vi "Test Strict Ambiguous ISO8601 Strings.vi"(8 "error in (no error)":errorcluster) -> (0 "error out":errorcluster)   [LabVIEW 2013]
uses:
  <vilib>/Utility/file.llb/Read From Spreadsheet File (string).vi
  <vilib>/addons/_JKI Toolkits/Caraya/classes/Assert/Assert False.vi
  <vilib>/addons/_JKI Toolkits/Caraya/classes/Assert/Assert True.vi
  <vilib>/addons/_JKI Toolkits/Caraya/classes/Assert/Assert.lvclass
  <vilib>/addons/_JKI Toolkits/Caraya/classes/Test/Test.lvclass
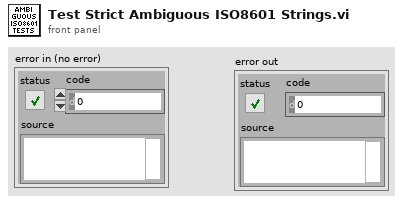
[diagram p1: front panel]
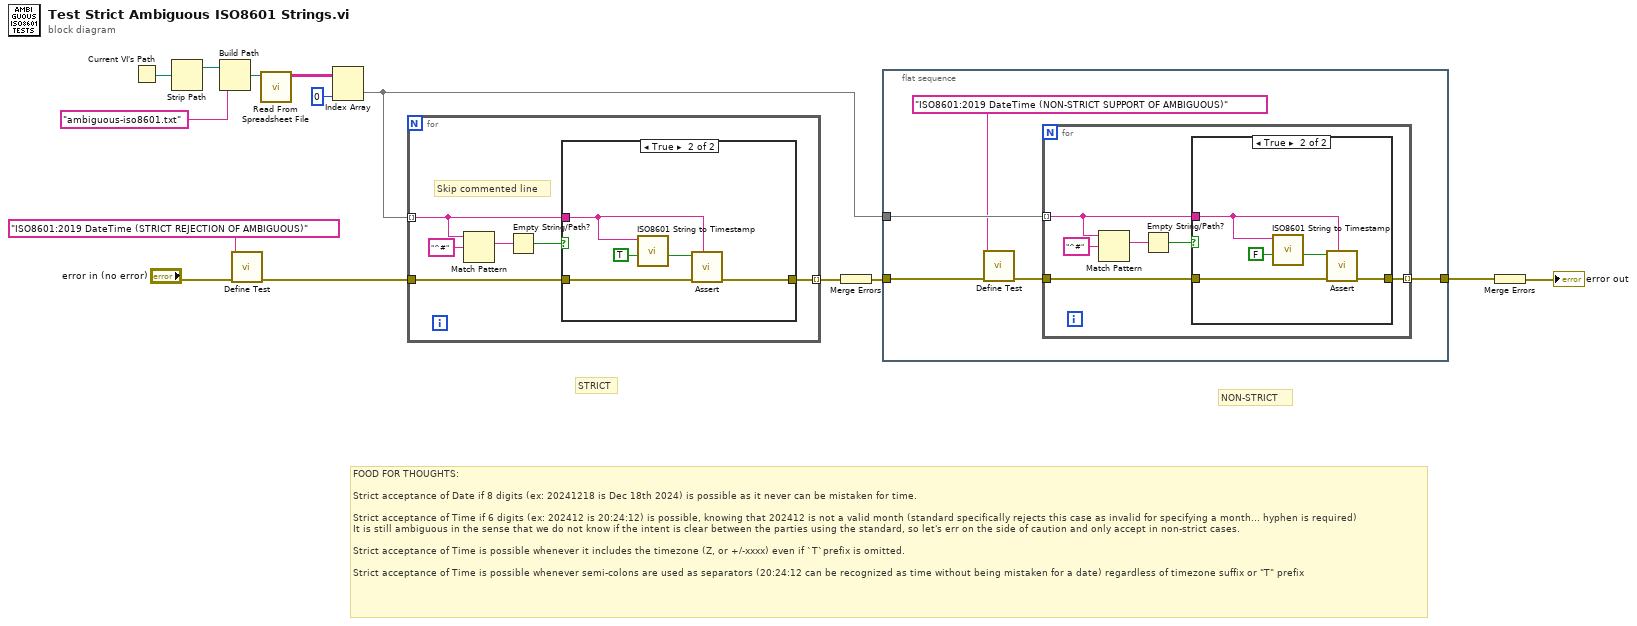
[diagram p0: block diagram]
diagram:
  # "NON-STRICT"
  # "STRICT"
  # "FOOD FOR THOUGHTS:\n\nStrict acceptance of Date if 8 digits (ex: 20241218 is Dec 18th 2024) is possible as it never can be mistaken for time.\n\nStrict acceptance of Time if 6 digits (ex: 202412 is 20:24:12) is possible, knowing that 202412 is not a valid month (standard specifically rejects this case as invalid for specifying a month... hyphen is required)\nIt is still ambiguous in the sense that we do not know if the intent is clear between the parties using the standard, so let's err on the side of caution and only accept in non-strict cases.\n\nStrict acceptance of Time is possible whenever it includes the timezone (Z, or +/-xxxx) even if `T`prefix is omitted.\n\nStrict acceptance of Time is possible whenever semi-colons are used as separators (20:24:12 can be recognized as time without being mistaken for a date) regardless of timezone suffix or \"T\" prefix"
  n1 = Current VI's Path() -> (path=w8:path)
  n2 = Strip Path(path=w8) -> (stripped path=w9:path)  [unwired: 1 out]
  n3 = Build Path(base path=w9, name or relative path="ambiguous-iso8601.txt") -> (appended path=w10:path)
  n4 = call <vilib>:"Define Test.vi"("error in (no error)"="error in (no error)", "Label (VI Title)"="ISO8601:2019 DateTime (STRICT REJECTION OF AMBIGUOUS)") -> ("error out"=w13:errorcluster)  [unwired: 8 in, 1 out]
  n5 = call-poly <vilib>:"Read From Spreadsheet File.vi"("file path (dialog if empty)"=w10) -> ("all rows"=w6:string[][])  [unwired: 6 in, 4 out]
  n6 = Index Array(array=w6, index (col)=0 ("disabled index (col)")) -> (element=w2:string[])  [unwired: 1 in]
  n7 = for {
    tunnel: w2 -> [w18] mode=indexing
    tunnel: [w19] -> w4 mode=indexing
    tunnel: w13 -> [w20]
    # "Skip commented line"
    n8 = Match Pattern(string=w18, regular expression="^#") -> (match substring=w16:string)  [unwired: 1 in, 3 out]
    n9 = Empty String/Path?(string/path=w16) -> (empty?=w15:bool)
    n10 = case shown="True" w15 {
      tunnel: w20 -> [w21 w26]
      tunnel: [w21 w25] -> w19
      tunnel: w18 -> [_ w22]
      frame False {
        # "Skip"
      }
      frame True {
        n11 = call "ISO8601 String to Timestamp.vi"("Strict ISO? (T)"=TRUE, "ISO8601 String"=w22) -> ("valid?"=w23:bool)  [unwired: 7 in, 2 out]
        n12 = call-poly <vilib>:"Assert.vi"("Label"=w22, "error in (no error)"=w26, "False?"=w23) -> ("error out"=w25:errorcluster)  [unwired: 7 in, 1 out]
      }
    }
  }
  n13 = Merge Errors(w4) -> (w3:errorcluster)
  n14 = flat-sequence {
    tunnel: w2 -> [w31]
    tunnel: [w30] -> w1
    tunnel: w3 -> [w28]
    frame #0 {
      n15 = call <vilib>:"Define Test.vi"("error in (no error)"=w28, "Label (VI Title)"="ISO8601:2019 DateTime (NON-STRICT SUPPORT OF AMBIGUOUS)") -> ("error out"=w27:errorcluster)  [unwired: 8 in, 1 out]
      n16 = for {
        tunnel: w31 -> [w35] mode=indexing
        tunnel: [w36] -> w30 mode=indexing
        tunnel: w27 -> [w37]
        n17 = Match Pattern(string=w35, regular expression="^#") -> (match substring=w33:string)  [unwired: 1 in, 3 out]
        n18 = Empty String/Path?(string/path=w33) -> (empty?=w32:bool)
        n19 = case shown="True" w32 {
          tunnel: w37 -> [w38 w43]
          tunnel: [w38 w42] -> w36
          tunnel: w35 -> [_ w39]
          frame False {
            # "Skip"
          }
          frame True {
            n20 = call "ISO8601 String to Timestamp.vi"("Strict ISO? (T)"=FALSE, "ISO8601 String"=w39) -> ("valid?"=w40:bool)  [unwired: 7 in, 2 out]
            n21 = call-poly <vilib>:"Assert.vi"("Label"=w39, "error in (no error)"=w43, "True?"=w40) -> ("error out"=w42:errorcluster)  [unwired: 7 in, 1 out]
          }
        }
      }
    }
  }
  n22 = Merge Errors(w1) -> (→"error out":errorcluster)
